vi "Is Supported Protocol Version.vi"(8 "error in":errorcluster, 11 "protocol version":string) -> (0 "error out":errorcluster, 3 "supported?":bool)   [LabVIEW 2020, in "MCP Server.lvlib"]
doc: "Checks a protocol version (the MCP-Protocol-Version request header) against all versions of Supported Protocol Versions.vi, modern and legacy. Which era a request belongs to is decided per request by params._meta, not here."
uses:
  MCP Server.lvlib
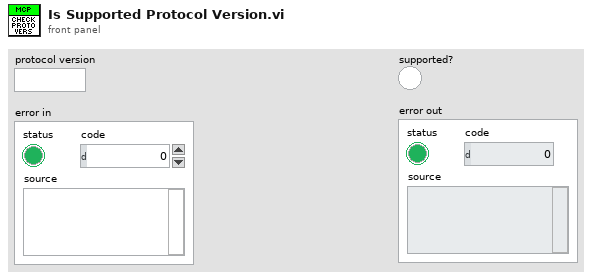
[diagram p1: front panel]
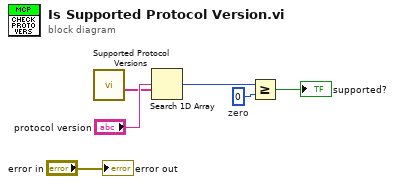
[diagram p0: block diagram]
diagram:
  w4 = 0  # zero
  n1 = call "Supported Protocol Versions.vi"() -> ("all versions"=w1:string[])  [unwired: 9 in, 2 out]
  n2 = Search 1D Array(1D array=w1, element="protocol version") -> (index of element=w5:i32)  [unwired: 1 in]
  n3 = Greater Or Equal?(x=w5, y=w4) -> (x >= y?=→"supported?":bool)
  "error out" <- "error in"
